vi "Cleanup Session.vi"(8 "error in":errorcluster, 11 "Plugin in":refnum<class "Modbus.lvclass">) -> (0 "error out":errorcluster, 3 "Plugin out":refnum<class "Modbus.lvclass">)   [LabVIEW 2026, in "Modbus.lvlib" / "Modbus.lvclass"]
uses:
  Modbus.lvclass
  <vilib>/ni/Modbus Library/API/Master/Modbus Master.lvclass
  Modbus.lvclass/Modbus.ctl
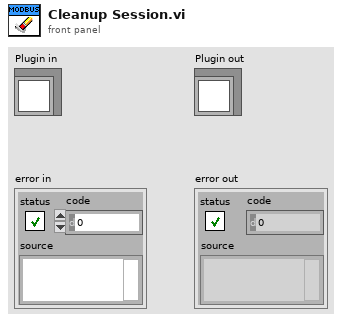
[diagram p1: front panel]
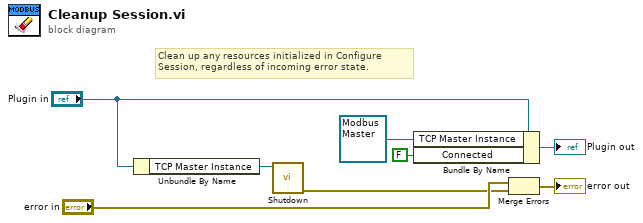
[diagram p0: block diagram]
diagram:
  # "Clean up any resources initialized in Configure Session, regardless of incoming error state."
  n1 = Unbundle By Name("Plugin in") -> ("TCP Master Instance"=w4:refnum<class "Modbus Master.lvclass">)
  n2 = call-dynamic "Shutdown.vi"("Modbus master in"=w4) -> ("error out"=w2:errorcluster)  [unwired: 10 in]
  n3 = Bundle By Name(cluster="Plugin in", "TCP Master Instance"=refnum<class "Modbus Master.lvclass"> refnum, "Connected"=FALSE) -> (→"Plugin out":refnum<class "Modbus.lvclass">)
  n4 = Merge Errors("error in", w2) -> (→"error out":errorcluster)
